vi "user32 GetWindowTextW.vi"(0 "hWnd":u64, 5 "nMaxCount":i32=256, 11 "error in":errorcluster) -> (4 "text":u16[](array[numeric]), 6 "return value":i32, 15 "error out":errorcluster)   [LabVIEW 2020, in "RemoteVI.lvlib"]
doc: "Returns the caption of the window hWnd through user32.dll GetWindowTextW (stdcall, called in any thread) as UTF-16 code units, so a caption in any language survives (narrowing it to LabVIEW bytes would not). The buffer is nMaxCount code units of zeros, and the caption is cut at its terminating 0. For a window of LabVIEW's own process the function sends WM_GETTEXT, which LabVIEW answers also while a dialog's modal loop runs (measured on LabVIEW 2025). return value is the number of characters copied, 0 for an empty caption or on failure. When error in carries an error the DLL is not called. Generated by scripts\\Build Win32 Wrappers.vi - do not edit by hand, rebuild it."
uses:
  RemoteVI.lvlib
  user32.dll
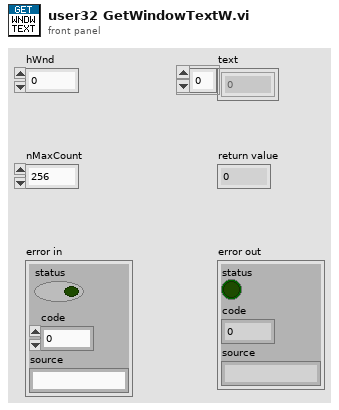
[diagram p1: front panel]
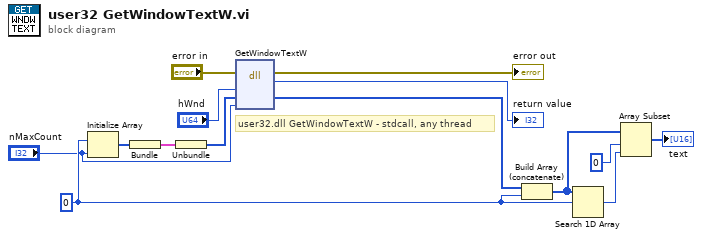
[diagram p0: block diagram]
diagram:
  w9 = u16 0
  # "user32.dll GetWindowTextW - stdcall, any thread"
  n1 = Initialize Array(w9, "nMaxCount") -> (w10:u16[])
  n2 = Bundle(w10) -> (w11:cluster{u16[]})  [unwired: 1 in]
  n3 = Unbundle(w11) -> (w2:u16[])
  n4 = dll-call lib="user32.dll" fn="GetWindowTextW"(error in="error in", "hWnd"="hWnd", "lpString"=w2, "nMaxCount"="nMaxCount") -> (error out=→"error out":errorcluster, →"return value":i32, "lpString"=w1:u16[])  [unwired: 4 in, 1 out]
  n5 = Build Array (concatenate)(w1, w9) -> (w12:u16[])
  n6 = Search 1D Array(1D array=w12, element=w9) -> (index of element=w13:i32)  [unwired: 1 in]
  n7 = Array Subset(array=w12, index=0, length=w13) -> (→"text":u16[])
